vi "Write Register.vi"(8 "error in (no error)":errorcluster, 9 "Value":u16, 10 "Register Address":u16, 11 "Modbus_Master in":refnum<class "Modbus_Master.lvclass">) -> (0 "error out":errorcluster, 3 "Modbus_Master out":refnum<class "Modbus_Master.lvclass">)   [LabVIEW 2021, in "Modbus_Master.lvclass"]
uses:
  Modbus_Master.lvclass
  Modbus_Master.lvclass/Modbus_Master.ctl
  <vilib>/NI/Modbus Library/API/Modbus API.lvclass/Modbus API.ctl
  <vilib>/NI/Modbus Library/Transmission Data Unit/Transmission Data Unit.lvclass/Transmission Data Unit.ctl
  <vilib>/NI/Modbus Library/Transmission Data Unit/Write Unit ID.vi
  <vilib>/NI/Modbus Library/API/Read Transmission Data Unit.vi
  <vilib>/NI/Modbus Library/API/Write Transmission Data Unit.vi
  <vilib>/NI/Modbus Library/API/Master/Modbus Master.lvclass
  C:/Program Files/National Instruments/LabVIEW 2021/vi.lib/NI/Modbus Library/API/Modbus API.lvclass
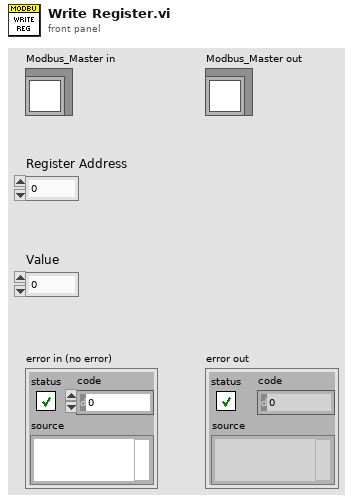
[diagram p1: front panel]
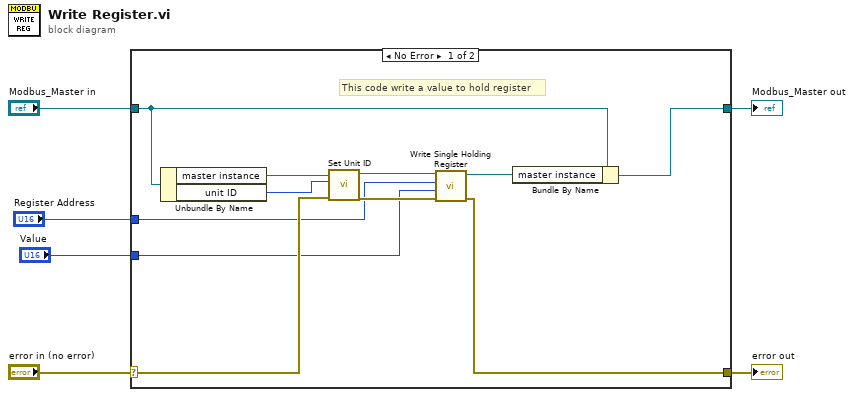
[diagram p0: block diagram]
diagram:
  n1 = case shown="No Error" "error in (no error)" {
    selector: "error in (no error)" -> [w15 w19]
    tunnel: [w10 w19] -> w5
    tunnel: [w8 w18] -> w3
    tunnel: "Modbus_Master in" -> [w9 w18]
    tunnel: "Register Address" -> [w12 _]
    tunnel: "Value" -> [w11 _]
    frame No Error {
      # "This code write a value to hold register"
      n2 = Unbundle By Name(w9) -> ("master instance"=w17:refnum<class "Modbus Master.lvclass">, "unit ID"=w16:u8)
      n3 = call <vilib>:"Set Unit ID.vi"("error in"=w15, "unit ID"=w16, "Modbus master in"=w17) -> ("error out"=w13:errorcluster, "Modbus master out"=w14:refnum<class "Modbus Master.lvclass">)  [unwired: 7 in]
      n4 = call-dynamic "Write Single Holding Register.vi"("error in"=w13, "register to write"=w11, "address"=w12, "Modbus master in"=w14) -> ("error out"=w10:errorcluster, "Modbus master out"=w7:refnum<class "Modbus Master.lvclass">)  [unwired: 6 in]
      n5 = Bundle By Name(cluster=w9, "master instance"=w7) -> (w8:refnum<class "Modbus_Master.lvclass">)
    }
    frame Error {
    }
  }
  "error out" <- w5
  "Modbus_Master out" <- w3
